vi "HistoryList.vi"(7 "Module Name":string="Module") -> ()   [LabVIEW 2017, in "DebugConsole.lvlib"]
uses:
  DebugConsole.lvlib
  _BroadcastDef.ctl
  508e9bfe-6490-4ffa-b47f-27ea34313f76.vi
  089f3262-7a84-4d39-9c60-bc06a6c67321.vi
  a9ada03b-0598-4474-9d19-b17bf33f6bd0.vi
  _csmlite/_PassAllowedMessage - Mapping.vi
  _Polymophic/CSM - Replace Marks in Messages.vi
  <vilib>/Utility/Data Type/Get Type Information.vi
  _csmHelper/lvcsmFile/lvcsm File Path.vi
  <vilib>/Utility/config.llb/Open Config Data.vi
  <vilib>/Utility/config.llb/Write Key.vi
  <vilib>/Utility/config.llb/Write Key (Boolean).vi
  <vilib>/Utility/Data Type/Get Array Information.vi
  <vilib>/Utility/config.llb/Get Key Names.vi
  <vilib>/Utility/config.llb/Remove Key.vi
  <vilib>/Utility/config.llb/Write Key (String).vi
  _csmHelper/lvcsmFile/Path to lvcsm String.vi
  <vilib>/Utility/config.llb/Write Key (I32).vi
  <vilib>/Utility/config.llb/Write Key (Double).vi
  <vilib>/Utility/config.llb/Close Config Data.vi
  _Polymophic/Add State(s) to Queue By BOOL(Element).vi
  <vilib>/Utility/config.llb/Read Key.vi
  <vilib>/Utility/config.llb/Read Key (Boolean).vi
  <vilib>/Utility/config.llb/Read Key (String).vi
  _csmHelper/lvcsmFile/lvcsm String to Path.vi
  <vilib>/Utility/config.llb/Read Key (I32).vi
  <vilib>/Utility/config.llb/Read Key (Double).vi
  _csmHelper/lvcsmFile/_Array of VData to VCluster.vi
  _csmlite/_csmlite.lvlib
  Communicable State Machine.lvlib
  _Shared/CSM Shared.lvlib
panel:
  in  "History":i32(listbox)
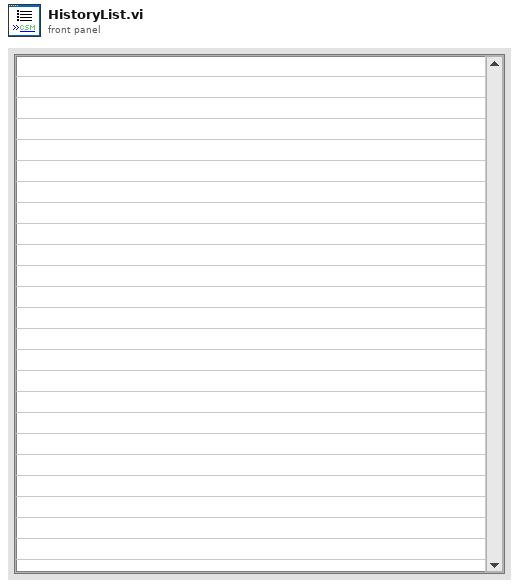
[diagram p1: front panel]
types:
  T1 = typedef "DebugConsole.lvlib/_BroadcastDef.ctl" = enum16{"<no action>", "Macro: Exit", "CSM: Module List Changed", "CSM: Scripts Changed", "CSM: Registration Changed", "CSM: Module Selected", "CSM: Message Excuted", "CSM: Broadcast Excuted", "CSM: Registration Action Excuted", "UI: Try to Change Command"}
  T2 = enum32{"Invalid", "Standard", "Closed", "Hidden", "Minimized", "Maximized"}
  T3 = enum32{"invalid app kind", "Development System", "Run Time System", "Student Edition", "Embedded LabVIEW", "Evaluation", "Custom"}
  T4 = cluster{"History Length":i32, "History":string[]}
  T5 = typedef "LVPoint32TypeDef.ctl" = cluster{"Horizontal":i32, "Vertical":i32}
  T6 = cluster{"Core":cluster{"Current VI Reference":refnum<vi>, "Close Panel on Exit?":bool}, "History Length":i32}
  T7 = cluster{"Current VI Reference":refnum<vi>, "Close Panel on Exit?":bool}
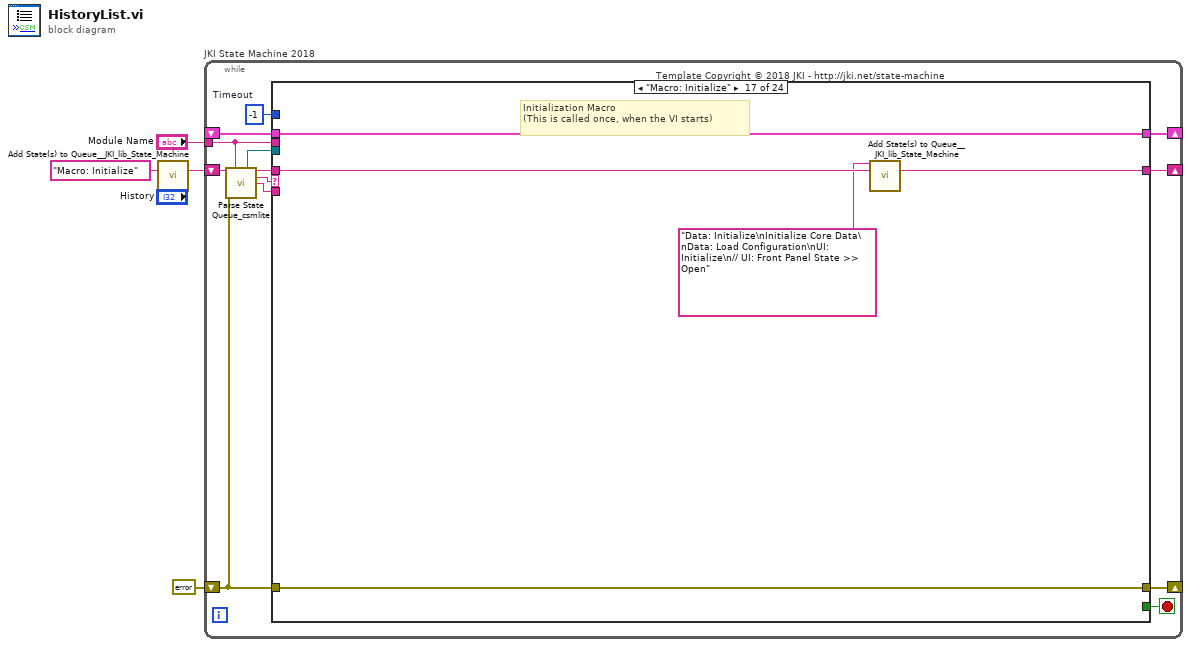
[diagram p0: block diagram]
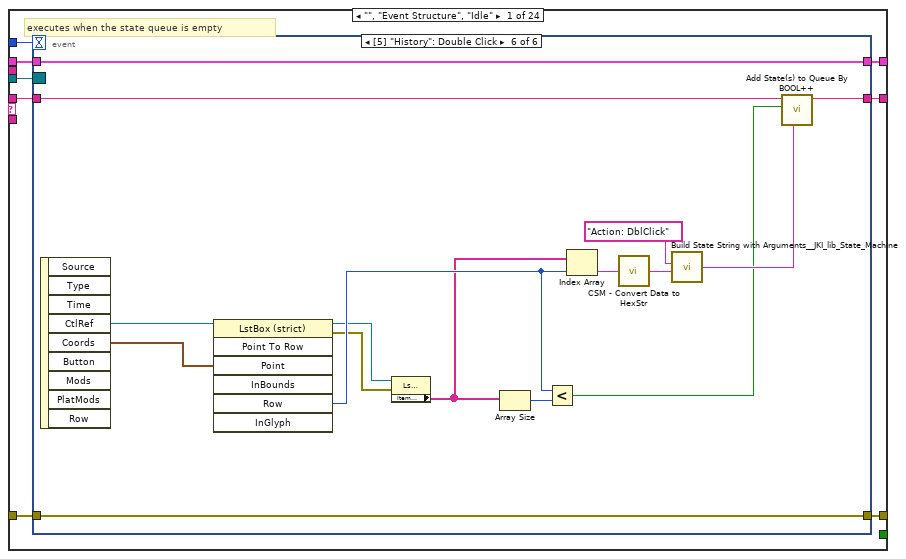
[diagram p2: hidden frame]
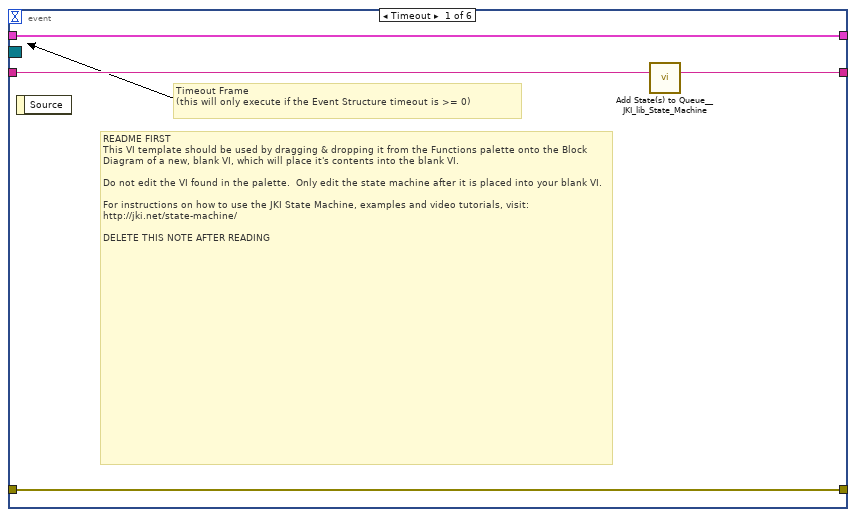
[diagram p3: hidden frame]
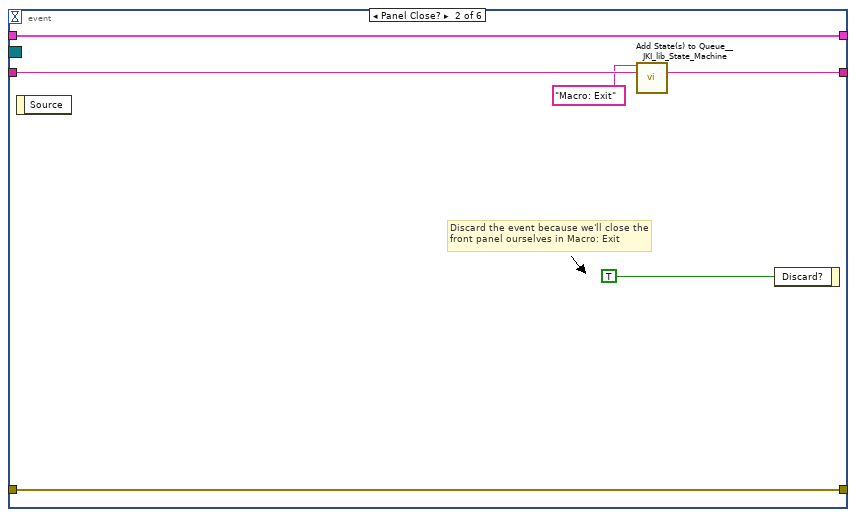
[diagram p4: hidden frame]
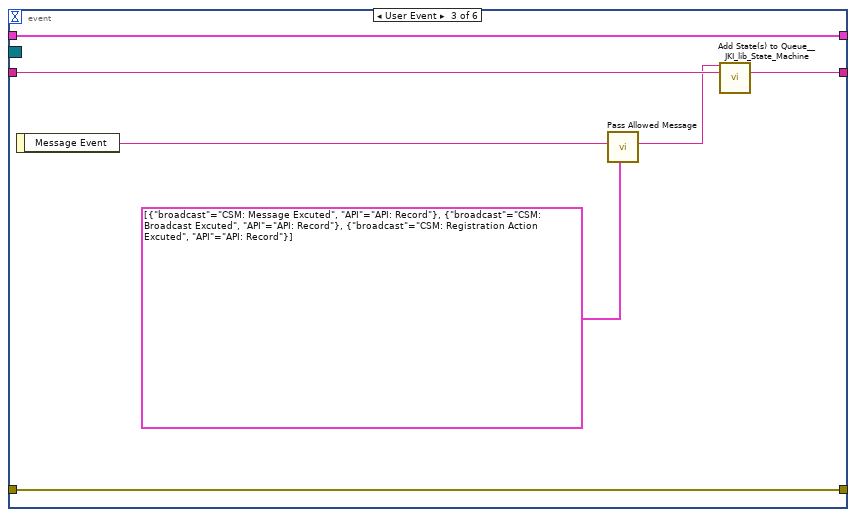
[diagram p5: hidden frame]
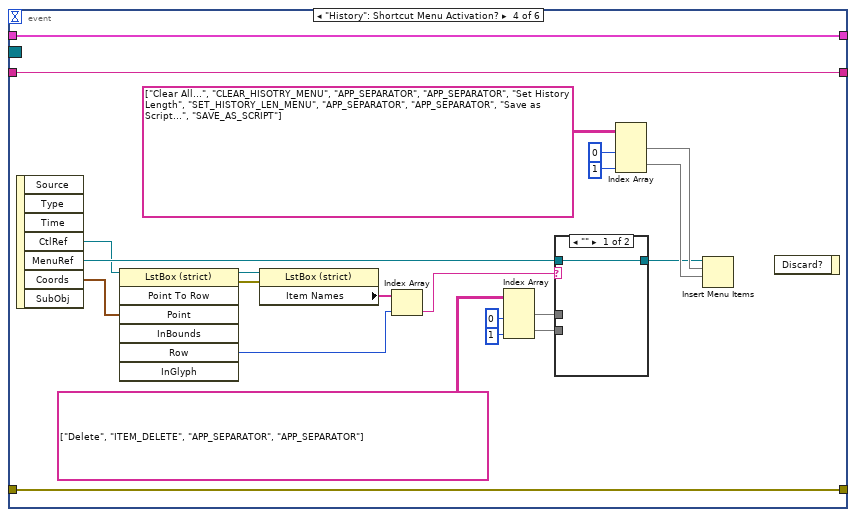
[diagram p6: hidden frame]
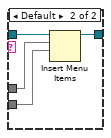
[diagram p7: hidden frame]
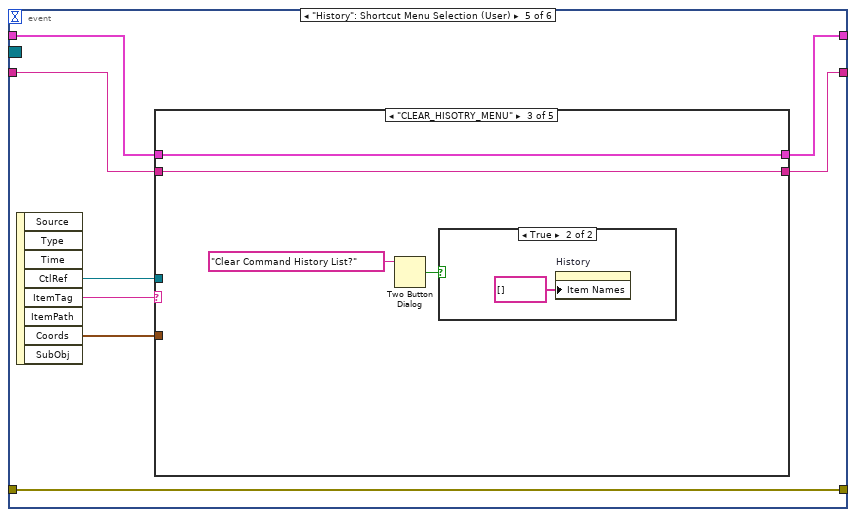
[diagram p8: hidden frame]
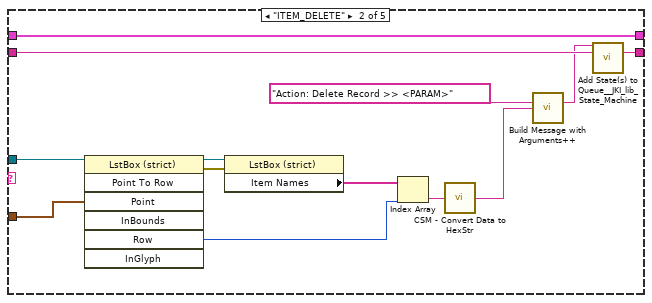
[diagram p10: hidden frame]
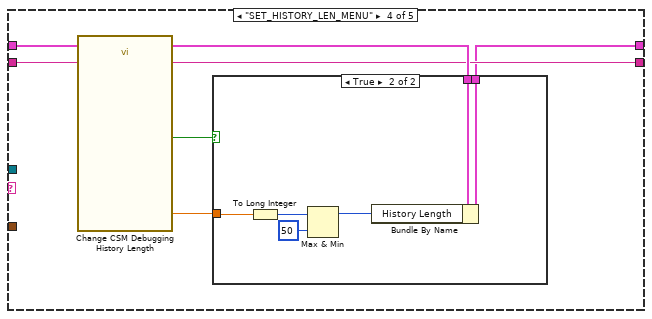
[diagram p12: hidden frame]
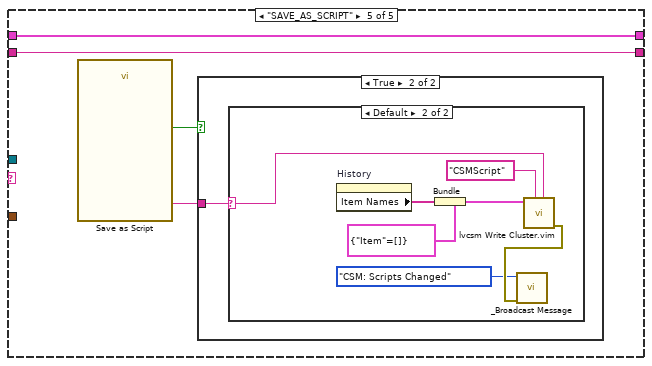
[diagram p14: hidden frame]
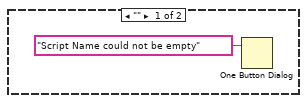
[diagram p16: hidden frame]
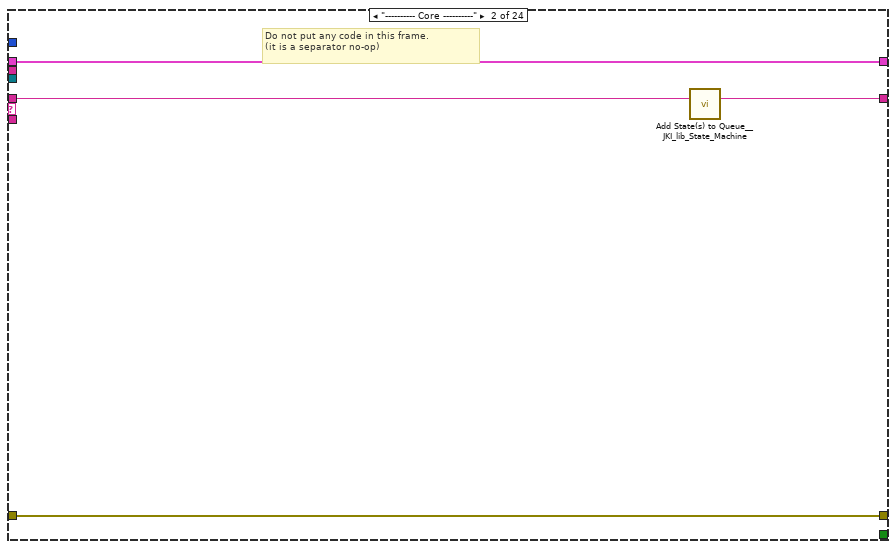
[diagram p17: hidden frame]
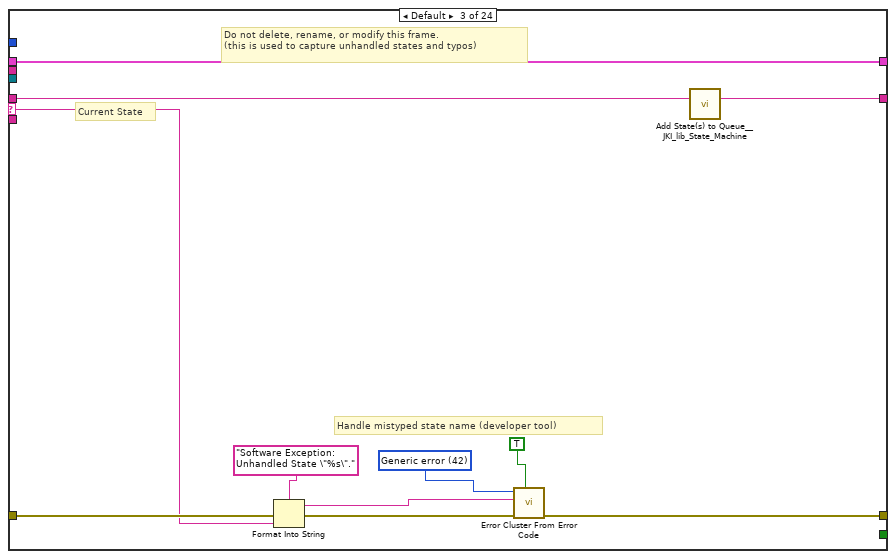
[diagram p18: hidden frame]
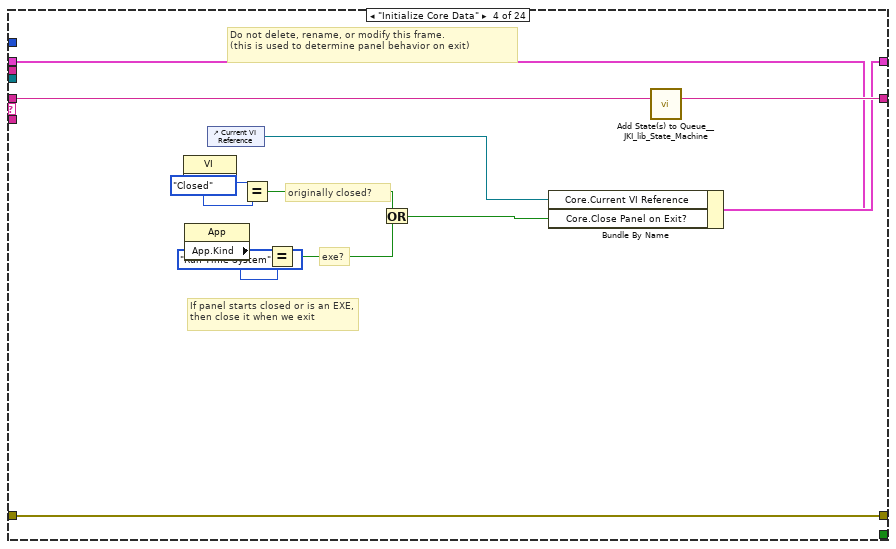
[diagram p19: hidden frame]
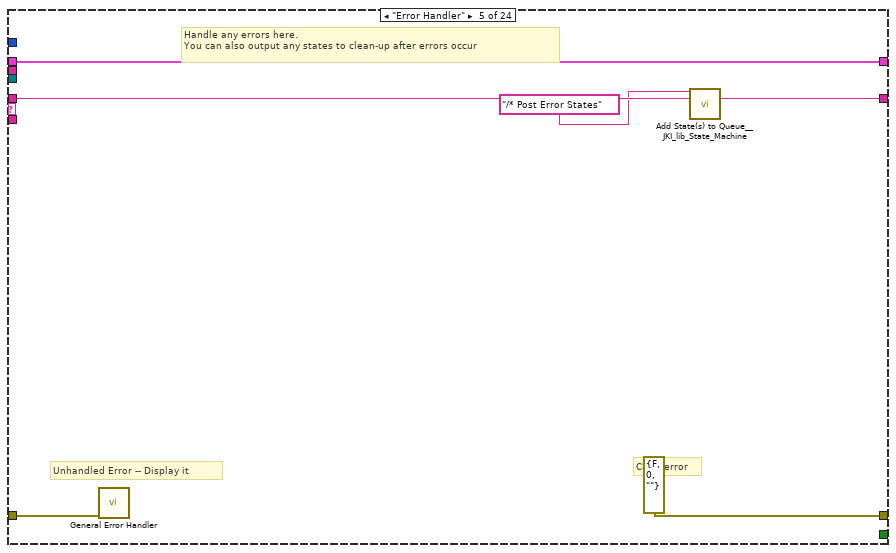
[diagram p20: hidden frame]
diagram:
  n1 = call <vilib>:"Add State(s) to Queue__JKI_lib_State_Machine.vi"("State(s) in (\"\")"="Macro: Initialize") -> ("States Out"=w3:string)  [unwired: 14 in]
  n2 = while "JKI State Machine 2018" {
    shift-right: [w10] -> _
    shift-left: _ -> [w9]
    shift-right: [w13] -> _
    shift-left: errorcluster {"status"=FALSE, "code"=0, "source"=""} ("error out") -> [w7]
    shift-right: [w12] -> _
    shift-left: w3 -> [w14]
    tunnel: "Module Name" -> [w5]
    stop <- w11 stop-if-true
    w8 = -1  # Timeout
    # "Template Copyright © 2018 JKI - http://jki.net/state-machine"
    n3 = call "Parse State Queue_csmlite.vi"("State Queue"=w14, "Current Module(\"\" to generate an ID)"=w5, "Error In (no error)"=w7) -> ("Event Registration Refnum"=w6:refnum<event-registration>, "Remaining States"=w16:string, "Current State"=w17:string, "Arguments"=w15:string)  [unwired: 9 in]
    n4 = case shown="\"Macro: Initialize\"" w17 {
      selector: w17 -> [_ _ w143 _ _ _ _ _ _ _ _ _ _ _ _ _ _ _ _ _ _ _ _ _]
      tunnel: w16 -> [w25 w142 w147 w166 w172 w177 w181 w187 w195 w203 w210 w214 w218 w224 w235 w304 w309 w319 w321 w326 w333 w339 w353 w369]
      tunnel: w15 -> [_ _ _ _ _ _ _ _ _ _ _ _ _ w219 w229 _ _ _ _ w323 _ w334 w352 w370]
      tunnel: w9 -> [w23 w139 w145 w159 w169 w175 w178 _ w194 w202 w205 w211 w216 w222 w231 w301 w306 w316 w320 w328 w330 w336 w342 w368]
      tunnel: [w22 w140 w149 w163 errorcluster {"status"=FALSE, "code"=0, "source"=""} ("error out") w174 w179 w184 w196 w204 w206 w212 w215 w220 w232 w302 w307 w317 w322 w329 w331 w337 w354 w371] -> w13
      tunnel: w7 -> [w21 w140 w148 w163 w168 w174 w179 w184 w196 w204 w207 w212 w215 w221 w233 w302 w307 w317 w322 w329 w331 w337 w354 w371]
      tunnel: [w24 w141 w146 w165 w171 w176 w180 w186 w195 w203 w209 w213 w217 w223 w234 w303 w308 w318 w321 w327 w332 w338 w353 w369] -> w12
      tunnel: [_ _ _ _ _ TRUE _ _ _ _ _ _ _ _ _ _ _ _ _ _ _ _ _ _] -> w11
      tunnel: [w20 w139 w145 w164 w169 w175 w178 w185 w191 w202 w205 w211 w216 w222 w231 w301 w306 w316 w320 w328 w330 w336 w342 w368] -> w10
      tunnel: w8 -> [w19 _ _ _ _ _ _ _ _ _ _ _ _ _ _ _ _ _ _ _ _ _ _ _]
      tunnel: w6 -> [w18 _ _ _ _ _ _ _ _ _ _ _ _ _ _ _ _ _ _ _ _ _ _ _]
      tunnel: w5 -> [_ _ _ _ _ _ _ _ w189 w199 _ _ _ _ _ _ _ _ _ _ _ _ _ _]
      frame "", "Event Structure", "Idle" {
        # "executes when the state queue is empty"
        n5 = event shown="[5] \"History\": Double Click" {
          selector: w18 -> [_ _ _ _ _ _]
          dyn-events: _ -> [_ _ _ _ _ _]
          timeout: w19 -> [_ _ _ _ _ _]
          tunnel: w25 -> [w29 w35 w40 w64 w73 w138]
          tunnel: [w28 w34 w38 w64 w72 w125] -> w24
          tunnel: w23 -> [w26 w32 w41 w62 w76 w136]
          tunnel: [w27 w33 w42 w63 w77 w137] -> w22
          tunnel: w21 -> [w27 w33 w42 w63 w77 w137]
          tunnel: [w26 w32 w41 w62 w75 w136] -> w20
          event Timeout {
            # "README FIRST\nThis VI template should be used by dragging & dropping it from the Functions palette onto the Block Diagram of a new, blank VI, which will place it's contents into the blank VI.\n\nDo not edit the VI found in the palette.  Only edit the state machine after it is placed into your blank VI.\n\nFor instructions on how to use the JKI State Machine, examples and video tutorials, visit:\nhttp://jki.net/state-machine/\n\nDELETE THIS NOTE AFTER READING"
            # "Timeout Frame\n(this will only execute if the Event Structure timeout is >= 0)"
            n6 = event-data() -> ()  [unwired: 1 in, 1 out]
            n7 = call <vilib>:"Add State(s) to Queue__JKI_lib_State_Machine.vi"("State(s) in (\"\")"=w29) -> ("States Out"=w28:string)  [unwired: 14 in]
          }
          event Panel Close? {
            # "Discard the event because we'll close the front panel ourselves in Macro: Exit"
            n8 = event-data() -> ()  [unwired: 1 in, 1 out]
            n9 = call <vilib>:"Add State(s) to Queue__JKI_lib_State_Machine.vi"("State(s) in Front (\"\")"="Macro: Exit", "State(s) in (\"\")"=w35) -> ("States Out"=w34:string)  [unwired: 13 in]
            n10 = event-data("Discard?"=TRUE) -> ()  [unwired: 1 in, 1 out]
          }
          event User Event {
            n11 = event-data() -> ("Message Event"=w39:string)  [unwired: 1 in]
            n12 = call-poly "Pass Allowed Message.vi"("Mapping"=cluster{"broadcast":string, "API":string}[] [{"broadcast"="CSM: Message Excuted", "API"="API: Record"}, {"broadcast"="CSM: Broadcast Excuted", "API"="API: Record"}, {"broadcast"="CSM: Registration Action Excuted", "API"="API: Record"}], "JKISM External Event"=w39) -> ("States"=w37:string)  [unwired: 7 in]
            n13 = call <vilib>:"Add State(s) to Queue__JKI_lib_State_Machine.vi"("State(s) in Front (\"\")"=w37, "State(s) in (\"\")"=w40) -> ("States Out"=w38:string)  [unwired: 13 in]
          }
          event "History": Shortcut Menu Activation? {
            n14 = event-data() -> ("CtlRef"=w46:refnum<vi>, "MenuRef"=w54:refnum<k9>, "Coords"=w45:T5)  [unwired: 1 in, 4 out]
            n15 = invoke class="LstBox (strict)" method="Point To Row"(reference=w46, "Point"=w45) -> (reference out=w47:refnum<vi>, error out=w43:errorcluster, "Row"=w44:i32)  [unwired: 5 in, 4 out]
            n16 = property class="LstBox (strict)"(reference=w47, error in=w43) -> ("Item Names"=w56:string[])  [unwired: 2 out]
            n17 = Index Array(array=w56, index=w44) -> (element=w48:string)
            n18 = Index Array(array=string[][] [["Delete", "ITEM_DELETE"], ["APP_SEPARATOR", "APP_SEPARATOR"]] ("item names"), index (col) #1=0 ("index (row)"), index (col) #2=1 ("index (row)")) -> (element #1=w51:string[], element #2=w49:string[])  [unwired: 2 in]
            n19 = case shown="\"\"" w48 {
              tunnel: [w65 w69] -> w55
              tunnel: w54 -> [w65 w68]
              tunnel: w51 -> [_ w67]
              tunnel: w49 -> [_ w66]
              frame "" {
              }
              frame Default {
                n20 = Insert Menu Items(7:w66, 8:w67, 9:w68) -> (3:w69:refnum<k9>)  [unwired: 3 in, 2 out]
              }
            }
            n21 = Index Array(array=string[][] [["Clear All...", "CLEAR_HISOTRY_MENU"], ["APP_SEPARATOR", "APP_SEPARATOR"], ["Set History Length", "SET_HISTORY_LEN_MENU"], ["APP_SEPARATOR", "APP_SEPARATOR"], ["Save as Script...", "SAVE_AS_SCRIPT"]] ("item names"), index (col) #1=0 ("index (row)"), index (col) #2=1 ("index (row)")) -> (element #1=w60:string[], element #2=w59:string[])  [unwired: 2 in]
            n22 = Insert Menu Items(7:w59, 8:w60, 9:w55) -> ()  [unwired: 3 in, 3 out]
            n23 = event-data() -> ()  [unwired: 2 in, 1 out]
          }
          event "History": Shortcut Menu Selection (User) {
            n24 = event-data() -> ("CtlRef"=w71:refnum<vi>, "ItemTag"=w74:string, "Coords"=w70:T5)  [unwired: 1 in, 5 out]
            n25 = case shown="\"CLEAR_HISOTRY_MENU\"" w74 {
              tunnel: w76 -> [w79 w92 w93 w102 w110]
              tunnel: [w78 w91 w95 w101 w113] -> w72
              tunnel: [w79 w92 w93 w100 w110] -> w75
              tunnel: w73 -> [w78 w90 w95 w101 w113]
              tunnel: w71 -> [_ w83 _ _ _]
              tunnel: w70 -> [_ w81 _ _ _]
              frame Default {
              }
              frame "ITEM_DELETE" {
                n26 = invoke class="LstBox (strict)" method="Point To Row"(reference=w83, "Point"=w81) -> (reference out=w85:refnum<vi>, error out=w84:errorcluster, "Row"=w80:i32)  [unwired: 5 in, 4 out]
                n27 = property class="LstBox (strict)"(reference=w85, error in=w84) -> ("Item Names"=w82:string[])  [unwired: 2 out]
                n28 = Index Array(array=w82, index=w80) -> (element=w87:string)
                n29 = call "CSM - Convert Data to HexStr.vi"("Variant"=w87) -> ("HEX String (0-9,A-F)"=w86:string)  [unwired: 8 in]
                n30 = call-poly "Build Message with Arguments++.vi"("States With Replace Token"="Action: Delete Record >> <PARAM>" ("State(s) in Front (\"\")"), "<param>"=w86) -> ("States"=w89:string)  [unwired: 13 in]
                n31 = call <vilib>:"Add State(s) to Queue__JKI_lib_State_Machine.vi"("State(s) in Front (\"\")"=w89, "State(s) in (\"\")"=w90) -> ("States Out"=w91:string)  [unwired: 13 in]
              }
              frame "CLEAR_HISOTRY_MENU" {
                n32 = Two Button Dialog(message="Clear Command History List?") -> (T button?=w94:bool)  [unwired: 2 in]
                n33 = case shown="True" w94 {
                  frame False {
                  }
                  frame True {
                    n34 = property on="History" class="LstBox (strict)"("Item Names"=string[] []) -> ()  [unwired: 2 in, 2 out]
                  }
                }
              }
              frame "SET_HISTORY_LEN_MENU" {
                n35 = call "Change CSM Debugging History Length"() -> ("History Length"=w99:dbl, "OK"=w98:bool)  [unwired: 17 in, 1 out]
                n36 = case shown="True" w98 {
                  tunnel: w102 -> [w103 w109]
                  tunnel: [w103 w108] -> w100
                  tunnel: w99 -> [_ w106]
                  frame False {
                  }
                  frame True {
                    n37 = To Long Integer(number=w106) -> (32bit integer=w104:i32)
                    n38 = Max & Min(x=w104, y=50) -> (max(x,y)=w107:i32)  [unwired: 1 out]
                    n39 = Bundle By Name(cluster=w109, "History Length"=w107) -> (w108:T6)
                  }
                }
              }
              frame "SAVE_AS_SCRIPT" {
                n40 = call "Save as Script"() -> ("Script"=w112:string, "OK"=w111:bool)  [unwired: 17 in, 1 out]
                n41 = case shown="True" w111 {
                  tunnel: w112 -> [_ w114]
                  frame False {
                  }
                  frame True {
                    n42 = case shown="Default" w114 {
                      selector: w114 -> [_ w121]
                      frame "" {
                        n43 = One Button Dialog(message="Script Name could not be empty") -> ()  [unwired: 1 in, 1 out]
                      }
                      frame Default {
                        n44 = property on="History" class="LstBox (strict)"() -> ("Item Names"=w120:string[])  [unwired: 2 in, 2 out]
                        n45 = Bundle(cluster=cluster{"Item":string[]} {"Item"=[]}, "Item"=w120) -> (w119:cluster{"Item":string[]})
                        n46 = call "lvcsm Write Cluster.vim"("Sub-section (\"\")"=w121, "Section"="CSMScript", "Configuration"=w119) -> ("error out"=w117:errorcluster)  [unwired: 8 in]
                        n47 = call "_Broadcast Message.vi"("Error in"=w117, "Broadcast"=_BroadcastDef."CSM: Scripts Changed") -> ()  [unwired: 9 in, 1 out]
                      }
                    }
                  }
                }
              }
            }
          }
          event "History": Double Click {
            n48 = event-data() -> ("CtlRef"=w127:refnum<vi>, "Coords"=w126:T5)  [unwired: 1 in, 7 out]
            n49 = invoke class="LstBox (strict)" method="Point To Row"(reference=w127, "Point"=w126) -> (reference out=w129:refnum<vi>, error out=w130:errorcluster, "Row"=w135:i32)  [unwired: 5 in, 4 out]
            n50 = property class="LstBox (strict)"(reference=w129, error in=w130) -> ("Item Names"=w132:string[])  [unwired: 2 out]
            n51 = Array Size(array=w132) -> (size(s)=w131:i32)
            n52 = Less?(x=w135, y=w131) -> (x < y?=w123:bool)
            n53 = Index Array(array=w132, index=w135) -> (element=w133:string)
            n54 = call "CSM - Convert Data to HexStr.vi"("Variant"=w133) -> ("HEX String (0-9,A-F)"=w134:string)  [unwired: 8 in]
            n55 = call <vilib>:"Build State String with Arguments__JKI_lib_State_Machine.vi"("Arguments (\"\")"=w134, "State"="Action: DblClick") -> ("State with Arguments"=w124:string)  [unwired: 4 in]
            n56 = call-poly "Add State(s) to Queue By BOOL++.vi"("TRUE (\"\")"=w124, "Condition"=w123, "State Queue (\"\")"=w138) -> ("Remaining States"=w125:string)  [unwired: 8 in]
          }
        }
      }
      frame "---------- Core ----------" {
        # "Do not put any code in this frame.\n(it is a separator no-op)"
        n57 = call <vilib>:"Add State(s) to Queue__JKI_lib_State_Machine.vi"("State(s) in (\"\")"=w142) -> ("States Out"=w141:string)  [unwired: 14 in]
      }
      frame Default {
        w152 = 42 items=["No error", "Argument error", "Memory is full", "Out of zone", "End of file", "File already open", "Generic file I/O error", "File not found", "File permission error", "Disk is full", "Duplicate path", "Too many files open", "System feature not enabled", "Resource file not found", "Cannot add resource", "Resource not found", "Image not found", "Image memory error", "Pen does not exist", "Config type invalid", "Config token not found", "Config parse error", "Config memory error", "Bad external code format", "Bad external code offset", "External code not present", "Null window", "Destroy window error", "Null menu", "Print aborted", "Bad print record", "Print driver error", "Windows error during printing", "Memory error during printing", "Print dialog error", "Generic print error", "Invalid device refnum", "Device not found", "Device parameter error", "Device unit error", "Cannot open device", "Device call aborted", "Generic error", "Cancelled by user", "Object ID too low", "Object ID too high", "Object not in heap", "Unknown heap", "Unknown object (invalid DefProc)", "Unknown object (DefProc not in table)", "Message out of range", "Invalid (null) method", "Unknown message", "Manager call not supported", "Bad address", "Network operation in progress", "Network operation timed out", "Connection is busy", "Network attribute not supported", "Network error", "Address in use", "System out of memory", "Connection aborted", "Connection refused", "Not connected", "Already connected", "Connection closed", "Initialization error (interapplication manager)", "Bad occurrence", "Wait on unbound occurrence handler", "Occurrence queue overflow", "Datalog type conflict", "Unused", "Unrecognized type (interapplication manager)", "Memory corrupt", "Failed to make temporary DLL", "Old CIN version", "Drag socket not found", "Failed to load drop-object", "Failed to register OLE object", "Failed to release OLE object", "Format specifier type mismatch", "Unknown format specifier", "Too few format specifiers", "Too many format specifiers", "Scan failed", "Newer CIN version", "Error converting to variant", "Runtime menu error", "Password tampered", "Variant attribute not found", "Incompatible variant data type", "Event data is not available", "Event Store is not present", "Occurrence is not found", "Event Queue is not created", "Event info is not available", "Refnum passed is NULL", "Error retrieving Class GUID", "Error retrieving CoClass GUID", "Error retrieving TypeLib GUID.", "Bad built application magic bytes.", "Specific driver is different from the specific driver associated with the Logical Name.", "There is no session opened to the class driver.", "Max Error", "MAX - Error with config objects", "MAX - Error loading configuration", "MAX - Group not supported"]
        # "Current State"
        # "Do not delete, rename, or modify this frame.\n(this is used to capture unhandled states and typos)"
        # "Handle mistyped state name (developer tool)"
        n58 = Format Into String(format string="Software Exception: Unhandled State \"%s\"." ("message"), error in=w148, w143) -> (resulting string=w151:string, error out=w150:errorcluster)  [unwired: 1 in]
        n59 = call <vilib>:"Error Cluster From Error Code.vi"("show call chain? (False)"=TRUE, "error in (no error)"=w150, "error message (\"\")"=w151, "error code (0)"=w152) -> ("error out"=w149:errorcluster)  [unwired: 5 in]
        n60 = call <vilib>:"Add State(s) to Queue__JKI_lib_State_Machine.vi"("State(s) in (\"\")"=w147) -> ("States Out"=w146:string)  [unwired: 14 in]
      }
      frame "Initialize Core Data" {
        # "Do not delete, rename, or modify this frame.\n(this is used to determine panel behavior on exit)"
        # "originally closed?"
        # "exe?"
        # "If panel starts closed or is an EXE, then close it when we exit"
        n61 = property class="VI"() -> ("FP.State"=w156:T2)  [unwired: 2 in, 2 out]
        n62 = property class="App"() -> ("App.Kind"=w162:T3)  [unwired: 2 in, 2 out]
        n63 = control-ref of="Current VI Reference"() -> (w157:refnum<vi>)
        n64 = Equal?(x=w156, y=T2."Closed" ("Front Panel Window:State")) -> (x = y?=w154:bool)
        n65 = Equal?(x=w162, y=T3."Run Time System" ("Application:Kind")) -> (x = y?=w160:bool)
        n66 = Or(x=w154, y=w160) -> (x .or. y?=w158:bool)
        n67 = Bundle By Name(cluster=w159, "Core.Current VI Reference"=w157, "Core.Close Panel on Exit?"=w158) -> (w164:T6)
        n68 = call <vilib>:"Add State(s) to Queue__JKI_lib_State_Machine.vi"("State(s) in (\"\")"=w166) -> ("States Out"=w165:string)  [unwired: 14 in]
      }
      frame "Error Handler" {
        # "Unhandled Error -- Display it"
        # "Handle any errors here.\nYou can also output any states to clean-up after errors occur"
        # "Clear error"
        n69 = call <vilib>:"General Error Handler.vi"("error in (no error)"=w168) -> ()  [unwired: 10 in, 5 out]
        n70 = call <vilib>:"Add State(s) to Queue__JKI_lib_State_Machine.vi"("State(s) in Front (\"\")"="/* Post Error States", "State(s) in (\"\")"=w172) -> ("States Out"=w171:string)  [unwired: 13 in]
      }
      frame "Exit" {
        # "Do not put any code in this frame.\n(No errors that occur here will be handled.)"
        n71 = call <vilib>:"Add State(s) to Queue__JKI_lib_State_Machine.vi"("State(s) in (\"\")"=w177) -> ("States Out"=w176:string)  [unwired: 14 in]
      }
      frame "---------- Data ----------" {
        # "Do not put any code in this frame.\n(It is a separator no-op. You can make a copy of this frame to create a new Data frame)"
        n72 = call <vilib>:"Add State(s) to Queue__JKI_lib_State_Machine.vi"("State(s) in (\"\")"=w181) -> ("States Out"=w180:string)  [unwired: 14 in]
      }
      frame "Data: Initialize" {
        w182 = 50  # History Length
        w183 = T7 {"Current VI Reference"=refnum, "Close Panel on Exit?"=FALSE}  # Core
        n73 = Bundle("Core"=w183, "History Length"=w182) -> (w185:T6)  [unwired: 1 in]
        n74 = call <vilib>:"Add State(s) to Queue__JKI_lib_State_Machine.vi"("State(s) in (\"\")"=w187) -> ("States Out"=w186:string)  [unwired: 14 in]
      }
      frame "Data: Load Configuration" {
        n75 = call "lvcsm Read Cluster.vim"("Section"=w189, "Default Prototype"=T4 {"History Length"=50, "History"=[]}) -> ("Cluster (Dup)"=w193:T4)  [unwired: 8 in, 1 out]
        n76 = Unbundle By Name(w193) -> ("History Length"=w190:i32, "History"=w188:string[])
        n77 = Bundle By Name(cluster=w194, "History Length"=w190) -> (w191:T6)
        n78 = property on="History" class="LstBox (strict)"("Item Names"=w188) -> ()  [unwired: 2 in, 2 out]
      }
      frame "Data: Save Configuration" {
        w197 = T4 {"History Length"=0, "History"=[]}  # cluster
        n79 = property on="History" class="LstBox (strict)"() -> ("Item Names"=w198:string[])  [unwired: 2 in, 2 out]
        n80 = Unbundle By Name(w202) -> ("History Length"=w201:i32)
        n81 = Bundle(cluster=w197, "History Length"=w201, "History"=w198) -> (w200:T4)
        n82 = call "lvcsm Write Cluster.vim"("Section"=w199, "Configuration"=w200) -> ()  [unwired: 9 in, 1 out]
      }
      frame "Data: Cleanup" {
        # "Cleanup any data and references, here.\n(this is called automatically, by the Macro: Exit)"
        n83 = Unbundle By Name(w205) -> ("Core.Current VI Reference"=w208:refnum<vi>)
        n84 = Close Reference(reference=w208, error in (no error)=w207) -> (error out=w206:errorcluster)
        n85 = call <vilib>:"Add State(s) to Queue__JKI_lib_State_Machine.vi"("State(s) in (\"\")"=w210) -> ("States Out"=w209:string)  [unwired: 14 in]
      }
      frame "---------- UI ----------" {
        # "Do not put any code in this frame.\n(It is a separator no-op. You can make a copy of this frame to create a new UI frame)"
        n86 = call <vilib>:"Add State(s) to Queue__JKI_lib_State_Machine.vi"("State(s) in (\"\")"=w214) -> ("States Out"=w213:string)  [unwired: 14 in]
      }
      frame "UI: Initialize" {
        # "Initialize the User Interface, here.\n(this is called automatically, by the Macro: Init)"
        n87 = call <vilib>:"Add State(s) to Queue__JKI_lib_State_Machine.vi"("State(s) in (\"\")"=w218) -> ("States Out"=w217:string)  [unwired: 14 in]
      }
      frame "UI: Cursor Set" {
        # "Argument"
        # "Set and Unset Cursor Busy.\n(Usage: \"UI: Cursor Set >> Busy|Idle\")"
        n88 = case shown="\"Idle\", Default" w219 {
          tunnel: w221 -> [w226 w228]
          tunnel: [w225 w227] -> w220
          frame "Idle", Default {
            n89 = call <vilib>:"Unset Busy.vi"("error in (no error)"=w226) -> ("error out"=w225:errorcluster)  [unwired: 10 in]
          }
          frame "Busy" {
            n90 = call <vilib>:"Set Busy.vi"("error in (no error)"=w228) -> ("error out"=w227:errorcluster)  [unwired: 9 in, 1 out]
          }
        }
        n91 = call <vilib>:"Add State(s) to Queue__JKI_lib_State_Machine.vi"("State(s) in (\"\")"=w224) -> ("States Out"=w223:string)  [unwired: 14 in]
      }
      frame "UI: Front Panel State" {
        # "Argument"
        # "Set Front Panel Open or Closed\n(Usage: \"UI: Front Panel State >> Open|Close\")"
        n92 = Unbundle By Name(w231) -> ("Core.Current VI Reference"=w230:refnum<vi>)
        n93 = case shown="\"Minimize\", \"Minimized\"" w229 {
          tunnel: w233 -> [w241 w256 w267 w280 w293]
          tunnel: [w243 w257 w269 w282 w295] -> w232
          tunnel: w230 -> [w242 w254 w268 w281 w294]
          frame "Open", "Standard", Default {
            w236 = T2."Standard" ("State")
            n94 = property class="VI"(reference=w242, error in=w241) -> (reference out=w239:refnum<vi>, error out=w240:errorcluster, "FP.State"=w238:T2)
            n95 = Not Equal?(x=w238, y=w236) -> (x != y?=w237:bool)
            n96 = case shown="True" w237 {
              tunnel: [w247 w249] -> w243
              tunnel: w240 -> [w246 w249]
              tunnel: w239 -> [w245 _]
              tunnel: w236 -> [w244 _]
              frame True {
                n97 = invoke class="VI" method="FP.Open"(reference=w245, error in=w246, "Activate"=TRUE, "State"=w244) -> (error out=w247:errorcluster)  [unwired: 1 in, 4 out]
              }
              frame False {
              }
            }
          }
          frame "Close", "Closed" {
            n98 = property class="VI"(reference=w254, error in=w256) -> (reference out=w253:refnum<vi>, error out=w255:errorcluster, "FP.State"=w251:T2)
            n99 = Not Equal?(x=w251, y=T2."Closed" ("Front Panel Window:State")) -> (x != y?=w250:bool)
            n100 = case shown="True" w250 {
              tunnel: [w258 w261] -> w257
              tunnel: w255 -> [w258 w260]
              tunnel: w253 -> [_ w259]
              frame False {
              }
              frame True {
                n101 = invoke class="VI" method="FP.Close"(reference=w259, error in=w260) -> (error out=w261:errorcluster)  [unwired: 1 in, 2 out]
              }
            }
          }
          frame "Hidden", "Hide" {
            w262 = T2."Hidden" ("State")
            n102 = property class="VI"(reference=w268, error in=w267) -> (reference out=w265:refnum<vi>, error out=w266:errorcluster, "FP.State"=w264:T2)
            n103 = Not Equal?(x=w264, y=w262) -> (x != y?=w263:bool)
            n104 = case shown="True" w263 {
              tunnel: [w273 w274] -> w269
              tunnel: w266 -> [w272 w274]
              tunnel: w265 -> [w271 _]
              tunnel: w262 -> [w270 _]
              frame True {
                n105 = invoke class="VI" method="FP.Open"(reference=w271, error in=w272, "State"=w270) -> (error out=w273:errorcluster)  [unwired: 2 in, 4 out]
              }
              frame False {
              }
            }
          }
          frame "Minimize", "Minimized" {
            w275 = T2."Minimized" ("State")
            n106 = property class="VI"(reference=w281, error in=w280) -> (reference out=w278:refnum<vi>, error out=w279:errorcluster, "FP.State"=w277:T2)
            n107 = Not Equal?(x=w277, y=w275) -> (x != y?=w276:bool)
            n108 = case shown="True" w276 {
              tunnel: [w286 w287] -> w282
              tunnel: w279 -> [w285 w287]
              tunnel: w278 -> [w284 _]
              tunnel: w275 -> [w283 _]
              frame True {
                n109 = invoke class="VI" method="FP.Open"(reference=w284, error in=w285, "State"=w283) -> (error out=w286:errorcluster)  [unwired: 2 in, 4 out]
              }
              frame False {
              }
            }
          }
          frame "Maximize", "Maximized" {
            w288 = T2."Maximized" ("State")
            n110 = property class="VI"(reference=w294, error in=w293) -> (reference out=w291:refnum<vi>, error out=w292:errorcluster, "FP.State"=w290:T2)
            n111 = Not Equal?(x=w290, y=w288) -> (x != y?=w289:bool)
            n112 = case shown="True" w289 {
              tunnel: [w299 w300] -> w295
              tunnel: w292 -> [w298 w300]
              tunnel: w291 -> [w297 _]
              tunnel: w288 -> [w296 _]
              frame True {
                n113 = invoke class="VI" method="FP.Open"(reference=w297, error in=w298, "State"=w296) -> (error out=w299:errorcluster)  [unwired: 2 in, 4 out]
              }
              frame False {
              }
            }
          }
        }
        n114 = call <vilib>:"Add State(s) to Queue__JKI_lib_State_Machine.vi"("State(s) in (\"\")"=w235) -> ("States Out"=w234:string)  [unwired: 14 in]
      }
      frame "---------- Macro ----------" {
        # "Do not put any code in this frame.\n(It is a separator no-op. You can make a copy of this frame to create a new Macro frame)"
        n115 = call <vilib>:"Add State(s) to Queue__JKI_lib_State_Machine.vi"("State(s) in (\"\")"=w304) -> ("States Out"=w303:string)  [unwired: 14 in]
      }
      frame "Macro: Initialize" {
        # "Initialization Macro\n(This is called once, when the VI starts)"
        n116 = call <vilib>:"Add State(s) to Queue__JKI_lib_State_Machine.vi"("State(s) in Front (\"\")"="Data: Initialize\nInitialize Core Data\nData: Load Configuration\nUI: Initialize\n// UI: Front Panel State >> Open", "State(s) in (\"\")"=w309) -> ("States Out"=w308:string)  [unwired: 13 in]
      }
      frame "Macro: Exit" {
        # "Exit Macro\n(This is called once, when the VI exits)"
        n117 = Unbundle By Name(w316) -> ("Core.Close Panel on Exit?"=w315:bool)
        n118 = Select(t="UI: Front Panel State >> Close", s=w315, f="") -> (s? t:f=w312:string)
        n119 = call <vilib>:"Add State(s) to Queue__JKI_lib_State_Machine.vi"("State(s) in (\"\")"=w312, "State(s) at Back (\"\")"="Data: Save Configuration\nData: Cleanup\nExit") -> ("States Out"=w310:string)  [unwired: 13 in]
        n120 = call <vilib>:"Add State(s) to Queue__JKI_lib_State_Machine.vi"("State(s) in Front (\"\")"=w310, "State(s) in (\"\")"=w319) -> ("States Out"=w318:string)  [unwired: 13 in]
      }
      frame "------------- API ---------------" {
      }
      frame "API: Record" {
        n121 = call-poly "Build Message with Arguments++.vi"("States With Replace Token"="Action: Record >> <param>" ("State(s) in Front (\"\")"), "<param>"=w323) -> ("States"=w325:string)  [unwired: 13 in]
        n122 = call <vilib>:"Add State(s) to Queue__jki_lib_state_machine.vi"("State(s) in Front (\"\")"=w325, "State(s) in (\"\")"=w326) -> ("States Out"=w327:string)  [unwired: 13 in]
      }
      frame "---------- New Category ----------" {
        # "Template Separator\n(You can make a copy of, or modify, this frame)"
        n123 = call <vilib>:"Add State(s) to Queue__JKI_lib_State_Machine.vi"("State(s) in (\"\")"=w333) -> ("States Out"=w332:string)  [unwired: 14 in]
      }
      frame "Action: DblClick" {
        # "Your code here.\n(You can make a copy of, or modify, this frame)"
        n124 = call "_Broadcast Message.vi"("Argument(\"\")"=w334, "Broadcast"=_BroadcastDef."UI: Try to Change Command") -> ()  [unwired: 9 in, 1 out]
        n125 = call <vilib>:"Add State(s) to Queue__JKI_lib_State_Machine.vi"("State(s) in (\"\")"=w339) -> ("States Out"=w338:string)  [unwired: 14 in]
      }
      frame "Action: Record" {
        n126 = call "CSM - Convert HexStr to Data.vi"("HEX String"=w352) -> ("Variant"=w350:variant)  [unwired: 7 in, 1 out]
        n127 = property on="History" class="LstBox (strict)"() -> ("Item Names"=w345:string[])  [unwired: 2 in, 2 out]
        n128 = Variant To Data(type="", Variant=w350) -> (data=w347:string)  [unwired: 1 in, 1 out]
        n129 = To Lower Case(string=w347) -> (all lower case string=w346:string)
        n130 = while {
          tunnel: w346 -> [w355]
          shift-right: [w358] -> w348
          shift-left: w345 -> [w359]
          stop <- w356 continue-if-true
          n131 = To Lower Case(string=w359) -> (all lower case string=w360:string[])
          n132 = Search 1D Array(1D array=w360, element=w355) -> (index of element=w357:i32)  [unwired: 1 in]
          n133 = Delete From Array(array=w359, index=w357) -> (array with subset deleted=w358:string[])  [unwired: 1 in, 1 out]
          n134 = Greater Or Equal To 0?(x=w357) -> (x >= 0?=w356:bool)
        }
        n135 = Build Array (concatenate)(w347, w348) -> (w351:string[])
        n136 = call "Remove Emptys From StrArray.vi"("Array In"=w351) -> ("Array Out"=w341:string[])  [unwired: 10 in]
        n137 = Unbundle By Name(w342) -> ("History Length"=w344:i32)
        n138 = Array Subset(array=w341, index=0, length=w344) -> (w340:string[])
        n139 = property on="History" class="LstBox (strict)"("Item Names"=w340) -> ()  [unwired: 2 in, 2 out]
      }
      frame "Action: Delete Record" {
        n140 = property on="History" class="LstBox (strict)"() -> ("Item Names"=w362:string[])  [unwired: 2 in, 2 out]
        n141 = call "CSM - Convert HexStr to Data.vi"("HEX String"=w370) -> ("Variant"=w367:variant)  [unwired: 7 in, 1 out]
        n142 = Variant To Data(type="", Variant=w367) -> (data=w364:string)  [unwired: 1 in, 1 out]
        n143 = To Lower Case(string=w364) -> (all lower case string=w363:string)
        n144 = while {
          tunnel: w363 -> [w372]
          shift-right: [w375] -> w365
          shift-left: w362 -> [w376]
          stop <- w373 continue-if-true
          n145 = To Lower Case(string=w376) -> (all lower case string=w377:string[])
          n146 = Search 1D Array(1D array=w377, element=w372) -> (index of element=w374:i32)  [unwired: 1 in]
          n147 = Delete From Array(array=w376, index=w374) -> (array with subset deleted=w375:string[])  [unwired: 1 in, 1 out]
          n148 = Greater Or Equal To 0?(x=w374) -> (x >= 0?=w373:bool)
        }
        n149 = call "Remove Emptys From StrArray.vi"("Array In"=w365) -> ("Array Out"=w361:string[])  [unwired: 10 in]
        n150 = property on="History" class="LstBox (strict)"("Item Names"=w361) -> ()  [unwired: 2 in, 2 out]
      }
    }
  }
